vi "Configure Module.vi"(8 "error in":errorcluster, 10 "IOV ref in":variant, 11 "9253 in":refnum<class "9253.lvclass">) -> (0 "error out":errorcluster, 2 "IOV ref out":variant, 3 "9253 out":refnum<class "9253.lvclass">)   [LabVIEW 2020, in "Modules.lvlib" / "9253.lvclass"]
uses:
  9253.lvclass
  <resource>/objmgr/cRIO.rc
  RSI Module/RSI Module.lvclass
  C:/Users/nitest/Desktop/Git 2020/niveristand-scan-engine-module-libraries/Source/RSI Module/RSI Module.lvclass
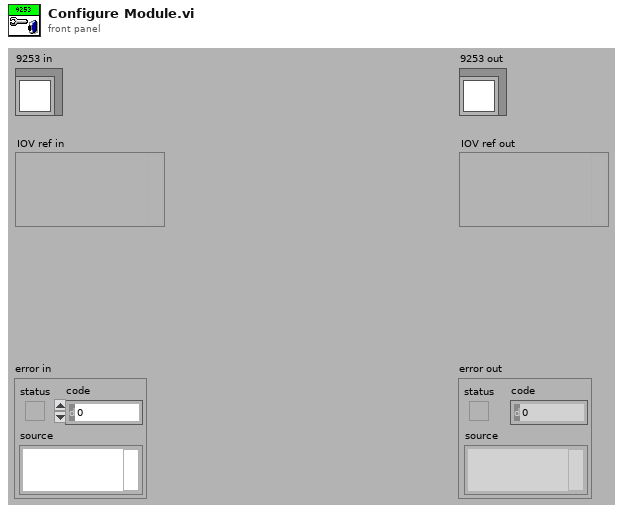
[diagram p1: front panel]
types:
  T1 = cluster{"fault detection enable":bool, "lower fault detection limit":dbl, "upper fault detection limit":dbl}[]
  T2 = typedef "Modules.lvlib/RSI Module.lvclass/Channels.ctl" = cluster{"# Input Channels":i32, "# Output Channels":i32, "Channel Type":T3, "Units":string}
  T3 = typedef "Modules.lvlib/RSI Module.lvclass/Channel Type.ctl" = enum16{"Analog", "Digital"}
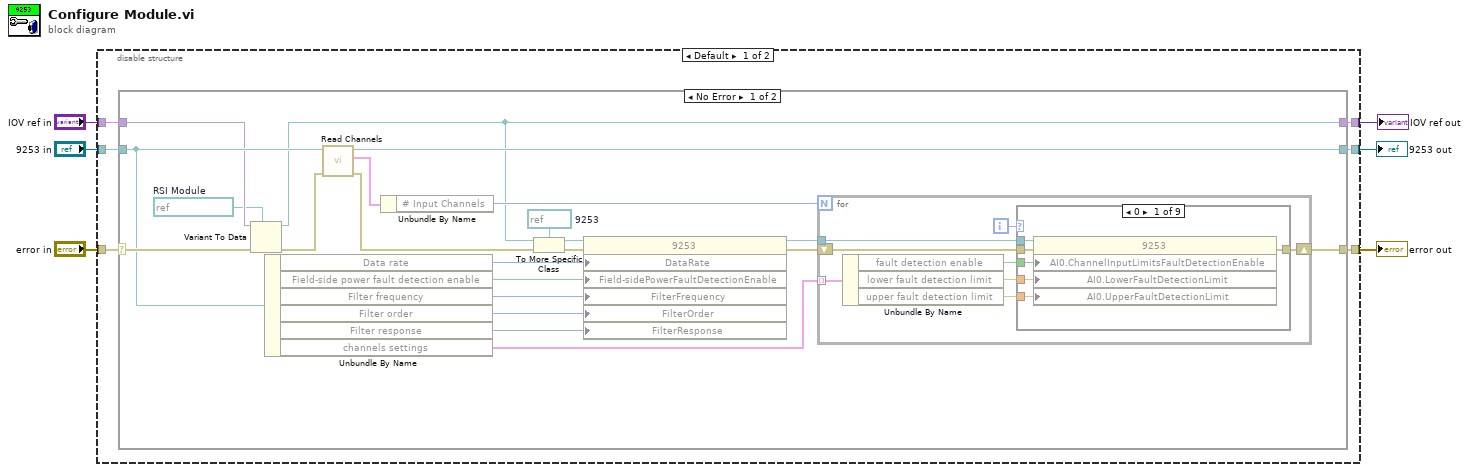
[diagram p0: block diagram]
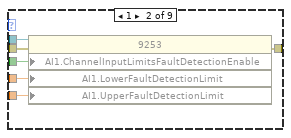
[diagram p2: hidden frame]
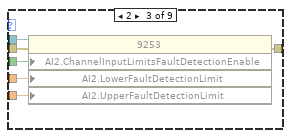
[diagram p3: hidden frame]
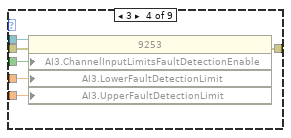
[diagram p4: hidden frame]
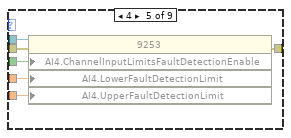
[diagram p5: hidden frame]
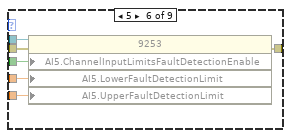
[diagram p6: hidden frame]
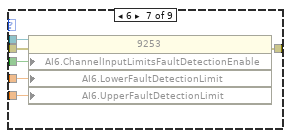
[diagram p7: hidden frame]
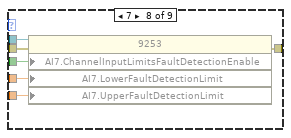
[diagram p8: hidden frame]
diagram:
  n1 = disable-structure shown="Default" {
    disable-tunnel: "error in" -> [w12 w97]
    disable-tunnel: [w11 w97] -> w5
    disable-tunnel: "9253 in" -> [w10 w96]
    disable-tunnel: [w9 w96] -> w3
    disable-tunnel: "IOV ref in" -> [w8 w95]
    disable-tunnel: [w7 w95] -> w1
    frame condition #0 {
      n2 = case shown="No Error" w12 {
        selector: w12 -> [w26 w94]
        tunnel: [w34 w94] -> w11
        tunnel: [w27 w93] -> w9
        tunnel: w10 -> [w22 w93]
        tunnel: w8 -> [w20 w92]
        tunnel: [w19 w92] -> w7
        frame No Error {
          w17 = refnum<k21> refnum  # 9253
          w18 = refnum<k21> refnum  # RSI Module
          n3 = Variant To Data(error in=w26, type=w18, Variant=w20) -> (data=w19:refnum<k21>, error out=w21:errorcluster)
          n4 = Unbundle By Name(w22) -> ("Data rate"=w33:u32, "Field-side power fault detection enable"=w32:bool, "Filter frequency"=w31:u32, "Filter order"=w30:u32, "Filter response"=w29:u32, "channels settings"=w28:T1)
          n5 = call "Read Channels.vi"("error in (no error)"=w21, "RSI Module in"=w22) -> ("error out"=w25:errorcluster, "Channels"=w24:T2, "RSI Module out"=w27:refnum<class "9253.lvclass">)  [unwired: 7 in]
          n6 = Unbundle By Name(w24) -> ("# Input Channels"=w23:i32)
          n7 = To More Specific Class(target class=w17, reference=w19, error in=w25) -> (specific class reference=w16:refnum<k21>, error out=w15:errorcluster)
          n8 = property class="9253"(reference=w16, error in=w15, "DataRate"=w33, "Field-sidePowerFaultDetectionEnable"=w32, "FilterFrequency"=w31, "FilterOrder"=w30, "FilterResponse"=w29) -> (reference out=w14:refnum<k21>, error out=w13:errorcluster)
          n9 = for {
            N: w23 -> [_]
            tunnel: w14 -> [w41]
            shift-right: [w42] -> w34
            shift-left: w13 -> [w40]
            tunnel: w28 -> [w38] mode=indexing
            i -> [w39]
            n10 = Unbundle By Name(w38) -> ("fault detection enable"=w37:bool, "lower fault detection limit"=w36:dbl, "upper fault detection limit"=w35:dbl)
            n11 = case shown="0" w39 {
              tunnel: [w48 w54 w60 w66 w72 w78 w84 w90 w91] -> w42
              tunnel: w37 -> [w47 w53 w59 w65 w71 w77 w83 w89 _]
              tunnel: w36 -> [w46 w52 w56 w62 w68 w74 w80 w86 _]
              tunnel: w35 -> [w45 w51 w55 w61 w67 w73 w79 w85 _]
              tunnel: w41 -> [w44 w50 w58 w64 w70 w76 w82 w88 _]
              tunnel: w40 -> [w43 w49 w57 w63 w69 w75 w81 w87 w91]
              frame 0 {
                n12 = property class="9253"(reference=w44, error in=w43, "AI0.ChannelInputLimitsFaultDetectionEnable"=w47, "AI0.LowerFaultDetectionLimit"=w46, "AI0.UpperFaultDetectionLimit"=w45) -> (error out=w48:errorcluster)  [unwired: 1 out]
              }
              frame 1 {
                n13 = property class="9253"(reference=w50, error in=w49, "AI1.ChannelInputLimitsFaultDetectionEnable"=w53, "AI1.LowerFaultDetectionLimit"=w52, "AI1.UpperFaultDetectionLimit"=w51) -> (error out=w54:errorcluster)  [unwired: 1 out]
              }
              frame 2 {
                n14 = property class="9253"(reference=w58, error in=w57, "AI2.ChannelInputLimitsFaultDetectionEnable"=w59, "AI2.LowerFaultDetectionLimit"=w56, "AI2.UpperFaultDetectionLimit"=w55) -> (error out=w60:errorcluster)  [unwired: 1 out]
              }
              frame 3 {
                n15 = property class="9253"(reference=w64, error in=w63, "AI3.ChannelInputLimitsFaultDetectionEnable"=w65, "AI3.LowerFaultDetectionLimit"=w62, "AI3.UpperFaultDetectionLimit"=w61) -> (error out=w66:errorcluster)  [unwired: 1 out]
              }
              frame 4 {
                n16 = property class="9253"(reference=w70, error in=w69, "AI4.ChannelInputLimitsFaultDetectionEnable"=w71, "AI4.LowerFaultDetectionLimit"=w68, "AI4.UpperFaultDetectionLimit"=w67) -> (error out=w72:errorcluster)  [unwired: 1 out]
              }
              frame 5 {
                n17 = property class="9253"(reference=w76, error in=w75, "AI5.ChannelInputLimitsFaultDetectionEnable"=w77, "AI5.LowerFaultDetectionLimit"=w74, "AI5.UpperFaultDetectionLimit"=w73) -> (error out=w78:errorcluster)  [unwired: 1 out]
              }
              frame 6 {
                n18 = property class="9253"(reference=w82, error in=w81, "AI6.ChannelInputLimitsFaultDetectionEnable"=w83, "AI6.LowerFaultDetectionLimit"=w80, "AI6.UpperFaultDetectionLimit"=w79) -> (error out=w84:errorcluster)  [unwired: 1 out]
              }
              frame 7 {
                n19 = property class="9253"(reference=w88, error in=w87, "AI7.ChannelInputLimitsFaultDetectionEnable"=w89, "AI7.LowerFaultDetectionLimit"=w86, "AI7.UpperFaultDetectionLimit"=w85) -> (error out=w90:errorcluster)  [unwired: 1 out]
              }
              frame Default {
              }
            }
          }
        }
        frame Error {
        }
      }
    }
    frame condition #1 (active) {
    }
  }
  "error out" <- w5
  "9253 out" <- w3
  "IOV ref out" <- w1
